vi "VIH ExtCmd - Params Store.vi"(7 "cmd (get)":enum16{"Init", "get", "set", "getcfg"}(ring)=enum."get", 10 "Params in":T1, 11 "Ext Command in":bool) -> (2 "Params":T1, 3 "Ext Command":bool)   [LabVIEW 2014]
doc: "::: VI Helpeks :::\nCopyright (c) 2000-2026 Konstantin Shifershteyn. All rights reserved."
panel:
  # "VI Helpeks\nCopyright (c) 2012-2026 Konstantin Shifershteyn"
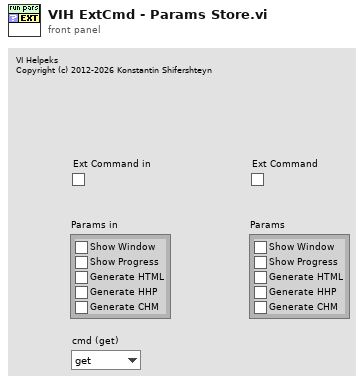
[diagram p1: front panel]
types:
  T1 = cluster{"Show Window":bool, "Show Progress":bool, "Generate HTML":bool, "Generate HHP":bool, "Generate CHM":bool}
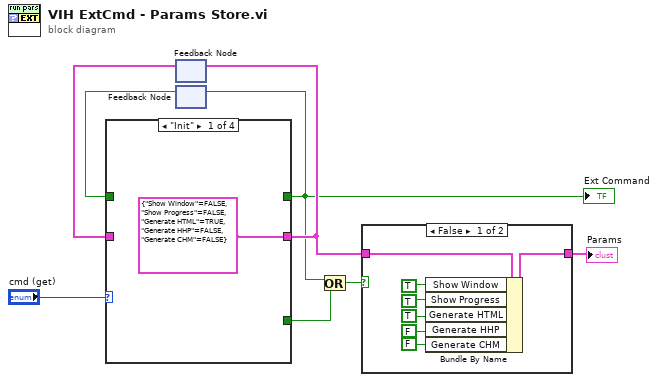
[diagram p0: block diagram]
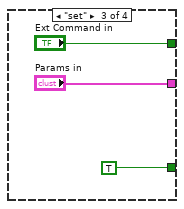
[diagram p4: hidden frame]
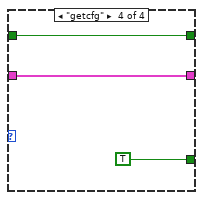
[diagram p5: hidden frame]
diagram:
  n1 = feedback #1() -> (w6:T1)  [unwired: 1 in]
  n2 = feedback #2() -> (w7:bool)  [unwired: 1 in]
  n3 = case shown="\"Init\"" "cmd (get)" {
    tunnel: [_ w11 "Ext Command in" w17] -> w3
    tunnel: [T1 {"Show Window"=FALSE, "Show Progress"=FALSE, "Generate HTML"=TRUE, "Generate HHP"=FALSE, "Generate CHM"=FALSE} ("Params in") w10 "Params in" w16] -> w5
    tunnel: w7 -> [_ w11 _ w17]
    tunnel: w6 -> [_ w10 _ w16]
    tunnel: [_ _ TRUE TRUE] -> w2
    frame "Init" {
    }
    frame "get" {
    }
    frame "set" {
    }
    frame "getcfg" {
    }
  }
  "Ext Command" <- w3
  n4 = feedback-in #1(w5) -> ()
  n5 = feedback-in #2(w3) -> ()
  n6 = Or(x=w3, y=w2) -> (x .or. y?=w1:bool)
  n7 = case shown="False" w1 {
    tunnel: w5 -> [w24 w25]
    tunnel: [w23 w25] -> w4
    frame False {
      n8 = Bundle By Name(cluster=w24, "Show Window"=TRUE, "Show Progress"=TRUE, "Generate HTML"=TRUE, "Generate HHP"=FALSE, "Generate CHM"=FALSE) -> (w23:T1)
    }
    frame True {
    }
  }
  "Params" <- w4
